vi "Cleanup.vi"(8 "error in (no error)":errorcluster, 11 "Node in":refnum<class "bt_Parallel_Threaded.lvclass">) -> (0 "error out":errorcluster, 3 "Node out":refnum<class "bt_Parallel_Threaded.lvclass">)   [LabVIEW 2021, in "BT.lvlib" / "bt_Parallel_Threaded.lvclass"]
uses:
  bt_Parallel_Threaded.lvclass
  bt_Parallel_Threaded.lvclass/bt_Parallel_Threaded.ctl
  System/bt_System.lvclass
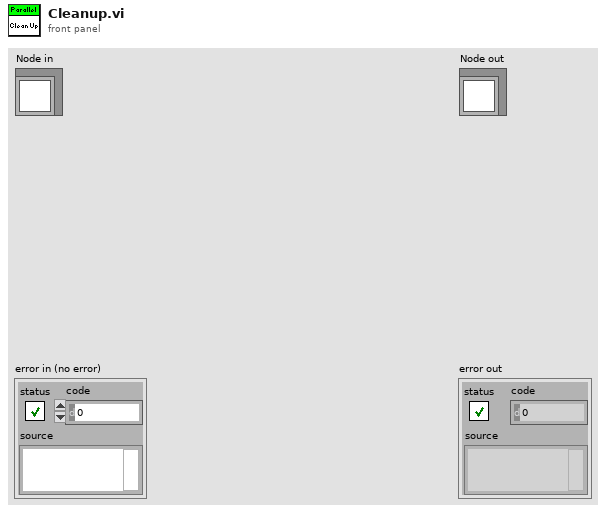
[diagram p1: front panel]
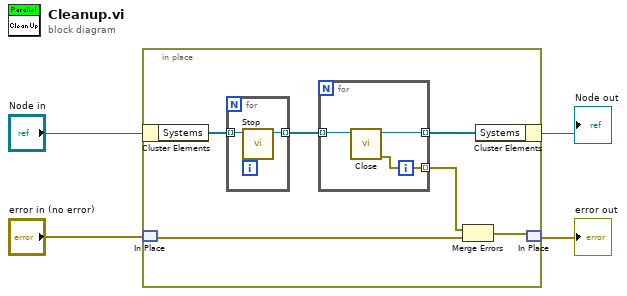
[diagram p0: block diagram]
diagram:
  n1 = in-place {
    n2 = in-place-cluster #1("Node in") -> ("Systems"=w7:refnum<class "bt_System.lvclass">[])
    n3 = in-place-match #2("error in (no error)") -> (w9:errorcluster)
    n4 = for {
      tunnel: w7 -> [w12] mode=indexing
      tunnel: [w11] -> w6 mode=indexing
      n5 = call "Stop.vi"("bt_System in"=w12) -> ("bt_System out"=w11:refnum<class "bt_System.lvclass">)  [unwired: 9 in, 1 out]
    }
    n6 = for {
      tunnel: [w15] -> w10 mode=indexing
      tunnel: [w13] -> w5 mode=indexing
      tunnel: w6 -> [w14] mode=indexing
      n7 = call-dynamic "Close.vi"("bt_System in"=w14) -> ("error out"=w13:errorcluster, "bt_System out"=w15:refnum<class "bt_System.lvclass">)  [unwired: 9 in]
    }
    n8 = Merge Errors(w5, w9) -> (w8:errorcluster)
    n9 = in-place-cluster #1("Systems"=w10) -> (→"Node out":refnum<class "bt_Parallel_Threaded.lvclass">)
    n10 = in-place-match #2(w8) -> (→"error out":errorcluster)
  }
